vi "LCDL Business Logic.vi"(8 "error in":errorcluster, 11 "CaptureDetectionLoopDataIn":T1={"Period"=-1, "Reset"=TRUE, "Iteration"=0, "Capture"=path "", "Mode"={"Replay"=enum."None", "Record"=enum."None"}, "Replay Run ID"="", "Frame Number"=0, "Core Module ID"=0, "EventRecorderLaunched"=FALSE, "Frame 0 relative seconds"=0.0, "Record Run ID"=""} {"Frame 0 relative seconds" format="%_19f"}) -> (0 "error out":errorcluster, 2 "Latest Frame":path, 3 "CaptureDetectionLoopDataOut":T1={"Period"=-1, "Reset"=TRUE, "Iteration"=0, "Capture"=path "", "Mode"={"Replay"=enum."None", "Record"=enum."None"}, "Replay Run ID"="", "Frame Number"=0, "Core Module ID"=0, "EventRecorderLaunched"=FALSE, "Frame 0 relative seconds"=0.0, "Record Run ID"=""} {"Frame 0 relative seconds" format="%_19f"})   [LabVIEW 2026, in "Launcher.lvlib"]
uses:
  Launcher.lvlib
  Capture detection loop data--cluster.ctl
  Mode.ctl
  ReplayMode.ctl
  RecordMode.ctl
panel:
  out "Trigger":bool
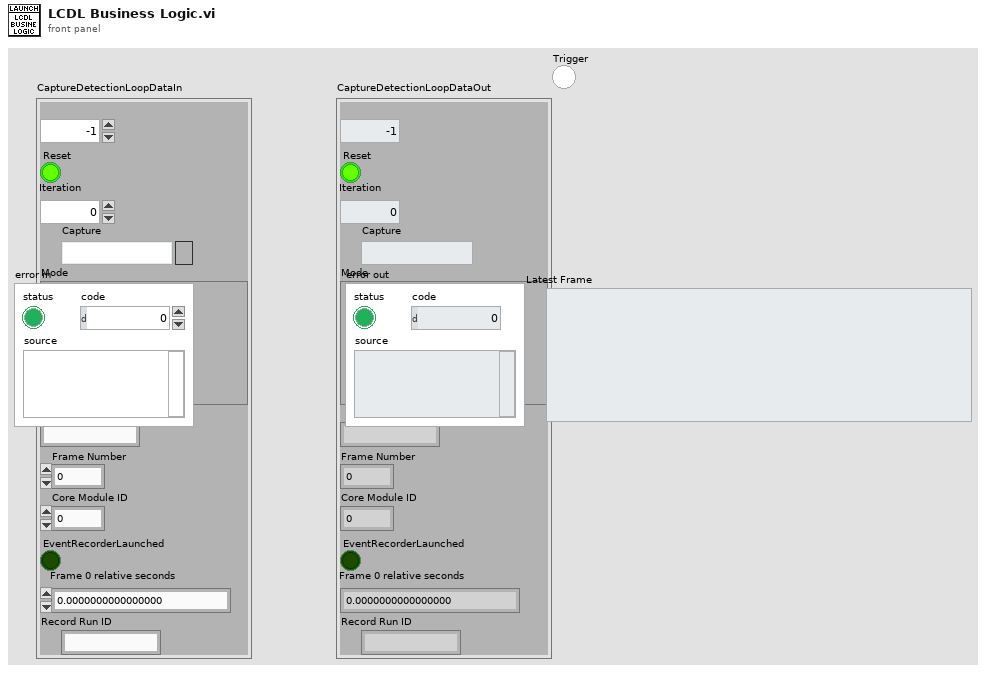
[diagram p1: front panel]
types:
  T1 = typedef "Capture detection loop data--cluster.ctl" = cluster{"Period":i32, "Reset":bool, "Iteration":i32, "Capture":path, "Mode":T2, "Replay Run ID":string, "Frame Number":u32, "Core Module ID":i32, "EventRecorderLaunched":bool, "Frame 0 relative seconds":dbl, "Record Run ID":string}
  T2 = typedef "Mode.ctl" = cluster{"Replay":T3, "Record":T4}
  T3 = typedef "ReplayMode.ctl" = enum16{"None", "User Events"}
  T4 = typedef "RecordMode.ctl" = enum16{"None", "User Events", "Benchmarks", "User Events and Benchmarks"}
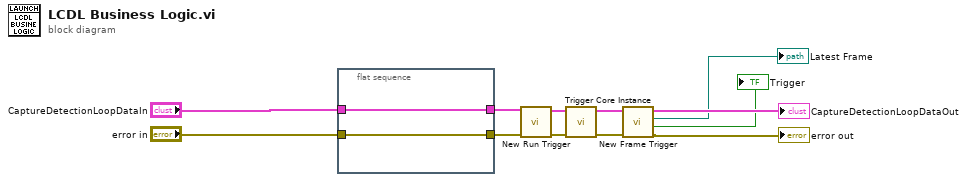
[diagram p0: block diagram]
diagram:
  n1 = flat-sequence {
    tunnel: "CaptureDetectionLoopDataIn" -> [w14]
    tunnel: [w14] -> w4
    tunnel: "error in" -> [w13]
    tunnel: [w13] -> w2
    frame #0 {
    }
  }
  n2 = call "New Run Trigger.vi"("error in"=w2, "CaptureDetectionLoopDataIn"=w4) -> ("error out"=w11:errorcluster, "CaptureDetectionLoopDataOut"=w12:T1)  [unwired: 7 in, 1 out]
  n3 = call "Trigger Core Instance.vi"("error in (no error)"=w11, "CaptureDetectionLoopDataIn"=w12) -> ("error out"=w9:errorcluster, "CaptureDetectionLoopDataOut"=w10:T1)  [unwired: 8 in]
  n4 = call "New Frame Trigger.vi"("error in"=w9, "CaptureDetectionLoopDataIn"=w10) -> ("error out"=→"error out":errorcluster, "Trigger"=→"Trigger":bool, "Latest Frame"=→"Latest Frame":path, "CaptureDetectionLoopDataOut"=→"CaptureDetectionLoopDataOut":T1)  [unwired: 6 in]
